vi "Find All Callers of State.vi"(8 "error in (no error)":errorcluster, 9 "State Name":string, 10 "Category (Optional)":string, 11 "JKI SM in":refnum<class "JKI SM.lvclass">) -> (0 "error out":errorcluster, 2 "Callers":T1(array[cluster]), 3 "JKI SM out":refnum<class "JKI SM.lvclass">)   [LabVIEW 2020, in "JKI State Machine API.lvlib" / "JKI SM.lvclass"]
uses:
  JKI SM.lvclass
  JKI SM.lvclass/JKI SM.ctl
  <vilib>/Utility/traverseref.llb/TRef TravTarget.ctl
  <userlib>/_OpenG.lib/string/string.llb/Trim Whitespace (String)__ogtk.vi
  <userlib>/_OpenG.lib/string/string.llb/openg_string.lvlib
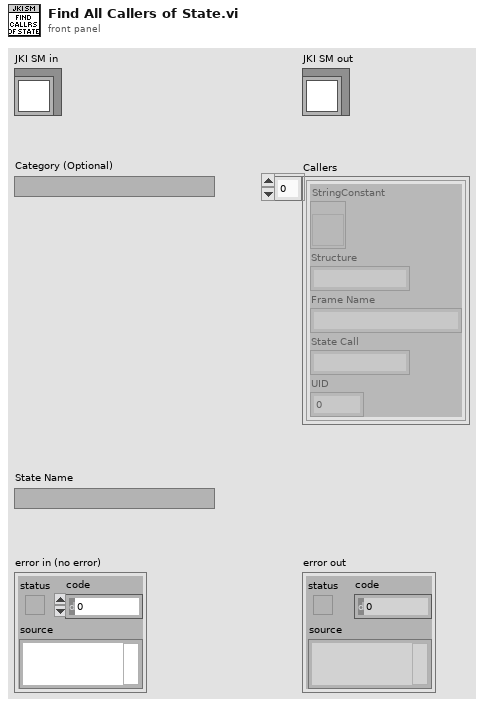
[diagram p1: front panel]
types:
  T1 = cluster{"StringConstant":refnum<vi>, "Structure":string, "Frame Name":string, "State Call":string, "UID":dbl}[]
  T2 = typedef "TRef TravTarget.ctl" = enum16{"FP", "BD", "Other"}
  T3 = cluster{"StringConstant":refnum<vi>, "Structure":string, "Frame Name":string, "State Call":string, "UID":i32}
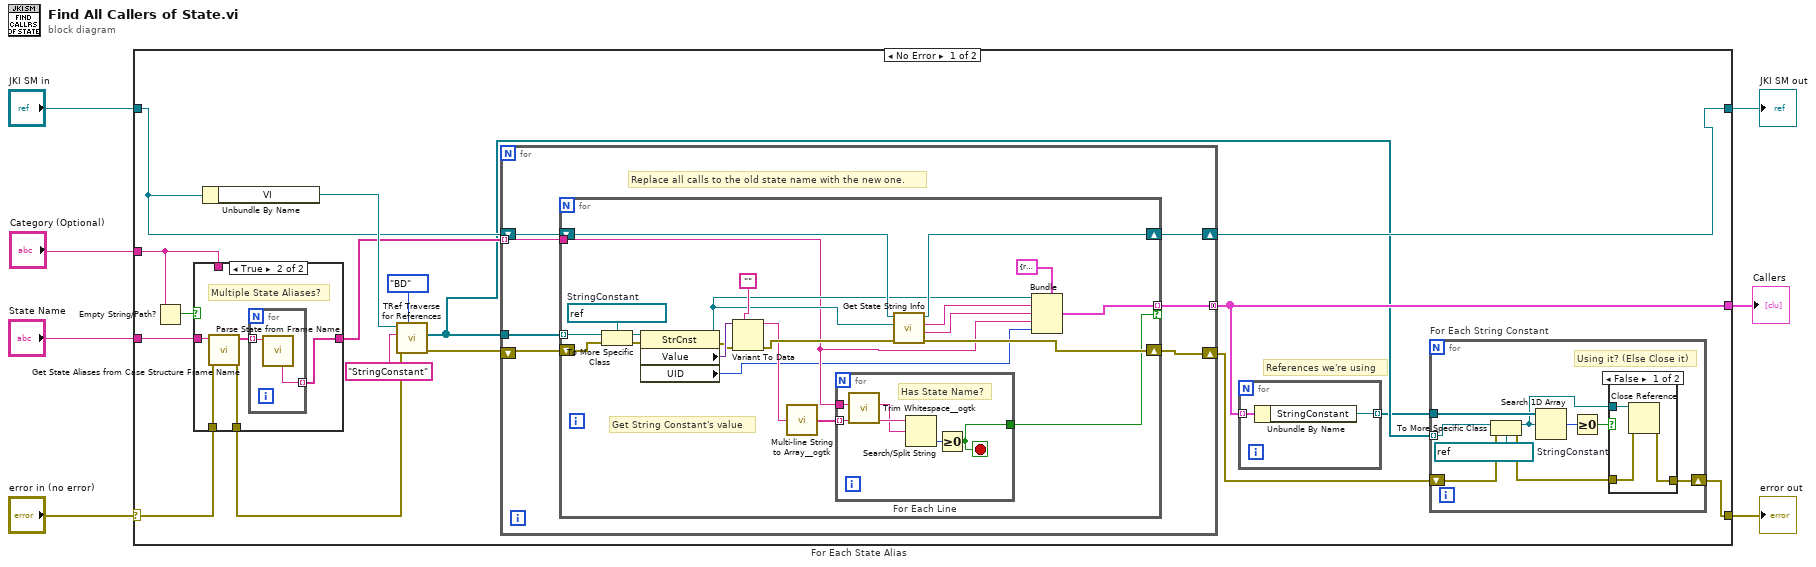
[diagram p0: block diagram]
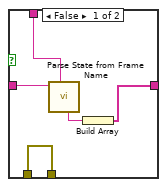
[diagram p3: hidden frame]
diagram:
  n1 = case shown="No Error" "error in (no error)" {
    selector: "error in (no error)" -> [w14 w87]
    tunnel: [w8 w87] -> w6
    tunnel: [w19 w86] -> w4
    tunnel: "JKI SM in" -> [w20 w86]
    tunnel: "State Name" -> [w17 _]
    tunnel: "Category (Optional)" -> [w16 _]
    tunnel: [w12 _] -> w1
    frame No Error {
      # "References we're using"
      n2 = Empty String/Path?(string/path=w16) -> (empty?=w15:bool)
      n3 = case shown="True" w15 {
        tunnel: [w41 w47] -> w18
        tunnel: w17 -> [w43 w49]
        tunnel: w16 -> [w42 _]
        tunnel: [w40 w46] -> w13
        tunnel: w14 -> [w40 w45]
        frame False {
          n4 = call "Parse State from Frame Name.vi"("Category (Optional)"=w42, "Frame or State Name"=w43) -> ("\"Category: State\" String"=w44:string)  [unwired: 4 in, 5 out]
          n5 = Build Array(w44) -> (w41:string[])
        }
        frame True {
          # "Multiple State Aliases?"
          n6 = call "Get State Aliases from Case Structure Frame Name.vi"("error in (no error)"=w45, "Frame or State Name"=w49) -> ("error out"=w46:errorcluster, "State Aliases"=w48:string[])  [unwired: 7 in, 1 out]
          n7 = for {
            tunnel: w48 -> [w51] mode=indexing
            tunnel: [w50] -> w47 mode=indexing
            n8 = call "Parse State from Frame Name.vi"("Frame or State Name"=w51) -> ("\"Category: State\" String"=w50:string)  [unwired: 5 in, 5 out]
          }
        }
      }
      n9 = Unbundle By Name(w20) -> ("VI"=w21:refnum<vi>)
      n10 = call <vilib>:"TRef Traverse for References.vi"("Traverse Target"=TRef_TravTarget."BD", "error in (no error)"=w13, "Class Name"="StringConstant", "VI Refnum"=w21) -> ("error out"=w22:errorcluster, "References"=w11:refnum<vi>[])  [unwired: 1 in, 5 out]
      n11 = for "For Each State Alias" {
        tunnel: w11 -> [w58]
        tunnel: [w53] -> w12 mode=concatenating
        tunnel: w18 -> [w52] mode=indexing
        shift-right: [w54] -> w9
        shift-left: w22 -> [w57]
        shift-right: [w55] -> w19
        shift-left: w20 -> [w56]
        # "Replace all calls to the old state name with the new one."
        n12 = for {
          tunnel: w58 -> [w80] mode=indexing
          tunnel: w52 -> [w60]
          shift-right: [w70] -> w55
          shift-left: w56 -> [w69]
          shift-right: [w71] -> w54
          shift-left: w57 -> [w77]
          tunnel: [w66] -> w53 mode=indexing if=w61
          w78 = refnum<vi> refnum  # StringConstant
          # "Get String Constant's value"
          n13 = To More Specific Class(target class=w78, reference=w80, error in=w77) -> (specific class reference=w79:refnum<vi>, error out=w76:errorcluster)
          n14 = property class="StrCnst"(reference=w79, error in=w76) -> (reference out=w68:refnum<vi>, error out=w72:errorcluster, "Value"=w75:variant, "UID"=w59:i32)
          n15 = Variant To Data(error in=w72, type="", Variant=w75) -> (data=w63:string, error out=w73:errorcluster)
          n16 = call <userlib>:"Multi-line String to Array__ogtk.vi"("string"=w63) -> ("lines"=w62:string[])
          n17 = for "For Each Line" {
            tunnel: w62 -> [w85] mode=indexing
            tunnel: w60 -> [w84]
            tunnel: [w82] -> w61
            stop <- w82 stop-if-true
            # "Has State Name?"
            n18 = call-poly <userlib>:"Trim Whitespace__ogtk.vi"("String in"=w84) -> ("String out"=w81:string)  [unwired: 6 in]
            n19 = Search/Split String(string=w85, search string/char (-)=w81) -> (offset of match=w83:i32)  [unwired: 1 in, 2 out]
            n20 = Greater Or Equal To 0?(x=w83) -> (x >= 0?=w82:bool)
          }
          n21 = call "Get State String Info.vi"("error in (no error)"=w73, "GObj Refnum in"=w68, "JKI SM in"=w69) -> ("error out"=w71:errorcluster, "Frame Name"=w64:string, "Structure"=w67:string, "JKI SM out"=w70:refnum<class "JKI SM.lvclass">)  [unwired: 5 in]
          n22 = Bundle(cluster=T3 {"StringConstant"=refnum, "Structure"="", "Frame Name"="", "State Call"="", "UID"=0}, "StringConstant"=w68, "Structure"=w67, "Frame Name"=w64, "State Call"=w60, "UID"=w59) -> (w66:T3)
        }
      }
      n23 = for {
        tunnel: w12 -> [w39] mode=indexing
        tunnel: [w38] -> w10 mode=indexing
        n24 = Unbundle By Name(w39) -> ("StringConstant"=w38:refnum<vi>)
      }
      n25 = for "For Each String Constant" {
        tunnel: w11 -> [w31] mode=indexing
        tunnel: w10 -> [w33]
        shift-right: [w25] -> w8
        shift-left: w9 -> [w27]
        w32 = refnum<vi> refnum  # StringConstant
        # "Using it? (Else Close it)"
        n26 = To More Specific Class(target class=w32, reference=w31, error in=w27) -> (specific class reference=w28:refnum<vi>, error out=w26:errorcluster)
        n27 = Search 1D Array(1D array=w33, element=w28) -> (index of element=w30:i32)  [unwired: 1 in]
        n28 = Greater Or Equal To 0?(x=w30) -> (x >= 0?=w29:bool)
        n29 = case shown="False" w29 {
          tunnel: w28 -> [w36 _]
          tunnel: [w35 w37] -> w25
          tunnel: w26 -> [w34 w37]
          frame False {
            n30 = Close Reference(reference=w36, error in (no error)=w34) -> (error out=w35:errorcluster)
          }
          frame True {
          }
        }
      }
    }
    frame Error {
    }
  }
  "error out" <- w6
  "JKI SM out" <- w4
  "Callers" <- w1
